vi "Shooter Teleop Handler.vi"() -> ()   [LabVIEW 2025]
uses:
  <vilib>/Rock Robotics/WPI/Joystick/XBox Axes Indexer.ctl
  <vilib>/Rock Robotics/WPI/Joystick/XBox Buttons Indexer.ctl
  Shooter/Implementation/Shooter Modes.ctl
  cc2de0f3-9757-4447-b84a-136412213354.vi
  cac903a5-6411-446e-9ddc-a5b591cf0002.vi
  08590b9f-08c0-4f10-921a-fd0bee2fbc93.vi
  627494dd-781a-424b-80dd-798a3808b72c.vi
  08f81d9b-c70a-4ca4-abda-0492c1fc3297.vi
  <vilib>/Rock Robotics/WPI/Utilities/WPI_GetSetVariantRefNum.vi
  Framework/Robot Global Data.vi
panel:
  in  "Purge Speeds":T1={"Transfer Speed"=-4600.0, "Kicker Speed"=0.95}
  in  "Ticks after shooting":dbl=10.0
  in  "Min Tick":dbl=20.0
  in  "Pre Transfer Speeds":T1={"Transfer Speed"=-1500.0, "Kicker Speed"=-0.4}
  in  "Oh Crap":cluster{"Hood Setpoint":dbl, "Flywheel":dbl}={"Hood Setpoint"=0.0, "Flywheel"=2000.0}
  in  "Tower":cluster{"Hood Setpoint":dbl, "Flywheel":dbl}={"Hood Setpoint"=3.5, "Flywheel"=2370.0}
  in  "A to A (no work)":cluster{"Hood Setpoint":dbl, "Flywheel":dbl}
  in  "C to A Far":cluster{"Hood Setpoint":dbl, "Flywheel":dbl}={"Hood Setpoint"=14.0, "Flywheel"=4600.0}
  in  "C to A Close":cluster{"Hood Setpoint":dbl, "Flywheel":dbl}={"Hood Setpoint"=15.0, "Flywheel"=3200.0}
  in  "Idle Speeds":cluster{"Hood Setpoint":dbl, "Flywheel":dbl}={"Hood Setpoint"=0.0, "Flywheel"=1000.0}
  in  "Transfer Speeds":T1={"Transfer Speed"=4600.0, "Kicker Speed"=0.95}
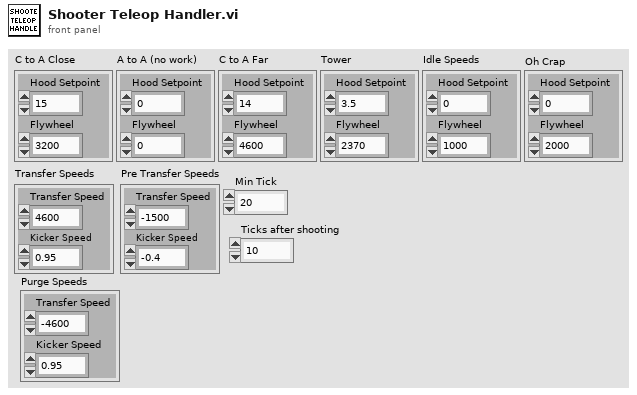
[diagram p1: front panel]
types:
  T1 = cluster{"Transfer Speed":dbl, "Kicker Speed":dbl}
  T2 = typedef "Shooter Modes.ctl" = enum16{"C to A Close", "C to A Far", "A to A", "Tower", "Interp", "Idle"}
  T3 = typedef "XBox Buttons Indexer.ctl" = enum16{"A", "B", "X", "Y", "Left Bumper", "Right Bumper", "Back", "Start", "Left Joystick", "Right Joystick"}
  T4 = typedef "XBox Axes Indexer.ctl" = enum16{"Left X", "Left Y", "Left Trigger", "Right Trigger", "Right X", "Right Y"}
  T5 = typedef "WPI_JoystickDevRef.ctl" = cluster{"Device":T6}
  T6 = typedef "WPI_JoystickDeviceEnum.ctl" = enum16{"USB 0", "USB 1", "USB 2", "USB 3", "USB 4", "USB 5"}
  T7 = cluster{"Hood Setpoint":dbl, "Flywheel Speed":dbl}
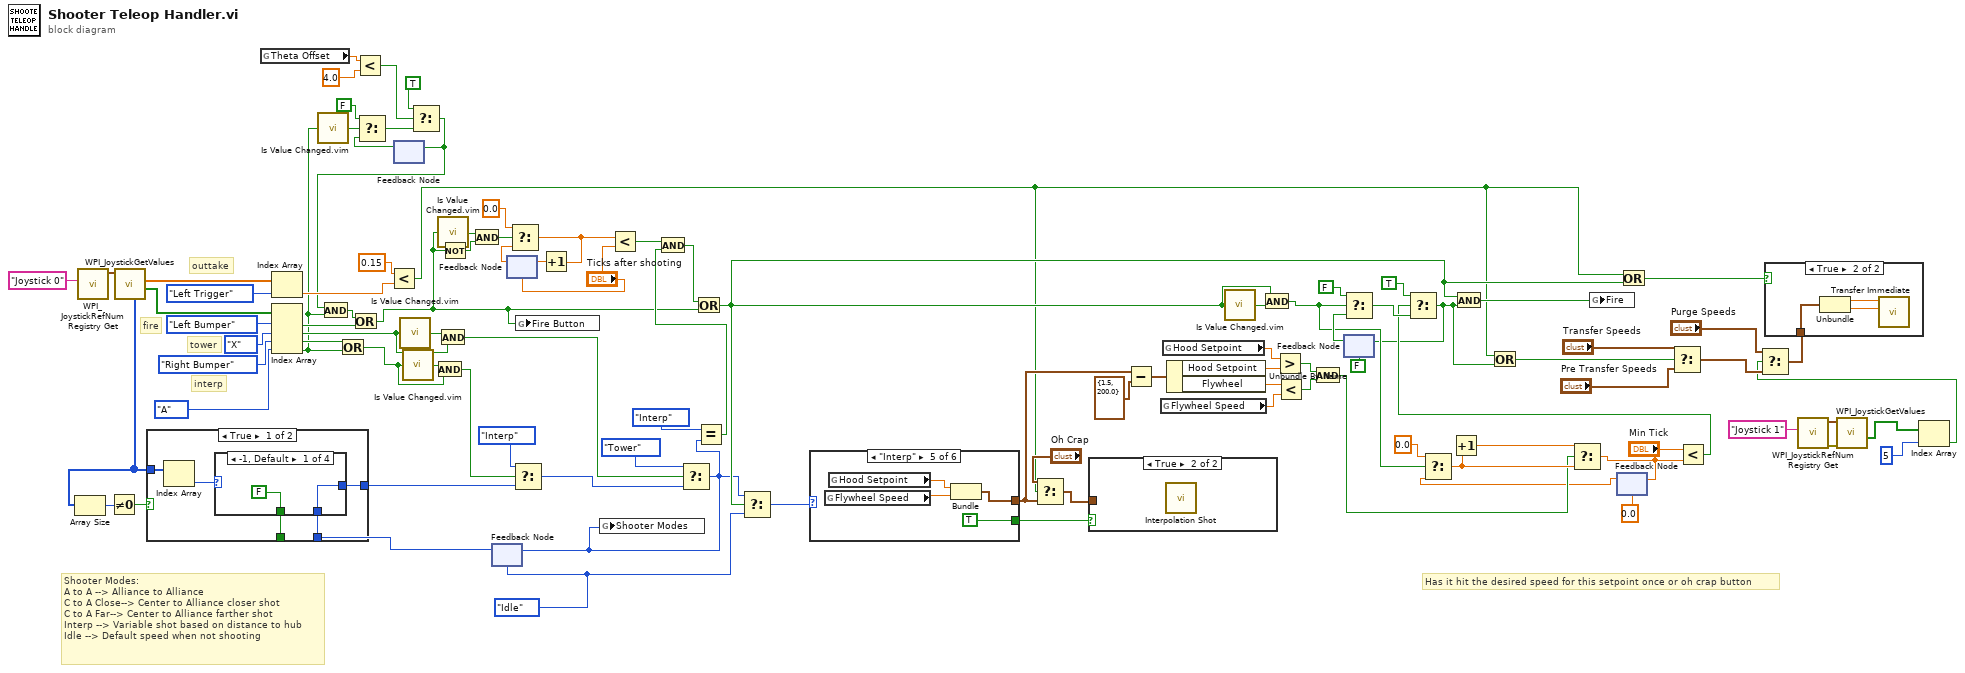
[diagram p0: block diagram]
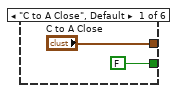
[diagram p3: hidden frame]
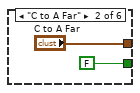
[diagram p4: hidden frame]
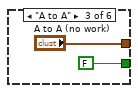
[diagram p5: hidden frame]
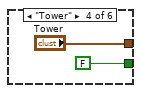
[diagram p6: hidden frame]
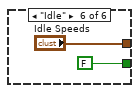
[diagram p7: hidden frame]
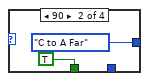
[diagram p8: hidden frame]
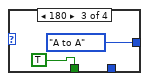
[diagram p9: hidden frame]
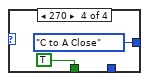
[diagram p10: hidden frame]
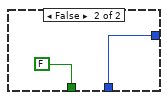
[diagram p11: hidden frame]
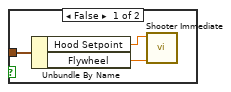
[diagram p12: hidden frame]
diagram:
  w64 = Shooter_Modes."Idle" ("Shooter Modes")
  # "interp"
  # "tower"
  # "Has it hit the desired speed for this setpoint once or oh crap button"
  # "Shooter Modes:\nA to A --> Alliance to Alliance\nC to A Close--> Center to Alliance closer shot\nC to A Far--> Center to Alliance farther shot\nInterp --> Variable shot based on distance to hub\nIdle --> Default speed when not shooting"
  # "outtake"
  # "fire"
  n1 = call <vilib>:"WPI_JoystickRefNum Registry Get.vi"("refnum name"="Joystick 0") -> ("JoystickDevRef"=w98:T5)  [unwired: 1 in, 9 out]
  n2 = call <vilib>:"WPI_JoystickGetValues.vi"("JoystickDevRef"=w98) -> ("Buttons"=w96:bool[], "Axes"=w97:dbl[], "POVs"=w77:i16[])  [unwired: 6 in, 2 out]
  n3 = Array Size(array=w77) -> (size(s)=w93:i32)
  n4 = Not Equal To 0?(x=w93) -> (x != 0?=w76:bool)
  n5 = global read "Robot Global Data.vi" "Theta Offset"() -> (w19:dbl)
  n6 = Index Array(array=w97, index=XBox_Axes_Indexer."Left Trigger" ("XBox Axes")) -> (element=w75:dbl)
  n7 = Index Array(array=w96, index #1=XBox_Buttons_Indexer."Left Bumper" ("XBox Buttons"), index #2=XBox_Buttons_Indexer."X" ("XBox Buttons"), index #3=XBox_Buttons_Indexer."Right Bumper" ("XBox Buttons"), index #4=XBox_Buttons_Indexer."A" ("XBox Buttons")) -> (element #1=w13:bool, element #2=w67:bool, element #3=w27:bool, element #4=w12:bool)
  n8 = call "Is Value Changed.vim"("value"=w12) -> ("changed or first call?"=w21:bool)
  n9 = Or(x=w27, y=w12) -> (x .or. y?=w26:bool)
  n10 = Less?(x=w19, y=4.0) -> (x < y?=w17:bool)
  n11 = Less?(x=0.15, y=w75) -> (x < y?=w23:bool)
  n12 = feedback #1() -> (w15:bool)  [unwired: 1 in]
  n13 = Select(t=FALSE, s=w21, f=w15) -> (s? t:f=w16:bool)
  n14 = call "Is Value Changed.vim"("value"=w67) -> ("changed or first call?"=w68:bool)
  n15 = call "Is Value Changed.vim"("value"=w26) -> ("changed or first call?"=w59:bool)
  n16 = Select(t=TRUE, s=w17, f=w16) -> (s? t:f=w10:bool)
  n17 = And(x=w10, y=w12) -> (x .and. y?=w11:bool)
  n18 = Or(x=w11, y=w13) -> (x .or. y?=w25:bool)
  n19 = feedback-in #1(w10) -> ()
  n20 = And(x=w59, y=w26) -> (x .and. y?=w58:bool)
  n21 = call "Is Value Changed.vim"("value"=w25) -> ("changed or first call?"=w41:bool)
  n22 = And(x=w68, y=w67) -> (x .and. y?=w65:bool)
  n23 = Not(x=w25) -> (.not. x?=w37:bool)
  n24 = And(x=w41, y=w37) -> (x .and. y?=w38:bool)
  n25 = feedback #2(w64) -> (w92:T2)
  n26 = case shown="True" w76 {
    tunnel: w77 -> [w104 _]
    tunnel: [w102 w114] -> w62
    tunnel: w92 -> [w101 w114]
    tunnel: [w100 FALSE ("changed or first call?")] -> _
    frame True {
      n27 = Index Array(array=w104) -> (element=w103:i16)  [unwired: 1 in]
      n28 = case shown="-1, Default" w103 {
        tunnel: [w106 Shooter_Modes."C to A Far" ("Shooter Modes") Shooter_Modes."A to A" ("Shooter Modes") Shooter_Modes."C to A Close" ("Shooter Modes")] -> w102
        tunnel: w101 -> [w106 _ _ _]
        tunnel: [FALSE ("changed or first call?") TRUE ("changed or first call?") TRUE ("changed or first call?") TRUE ("changed or first call?")] -> w100
        frame -1, Default {
        }
        frame 90 {
        }
        frame 180 {
        }
        frame 270 {
        }
      }
    }
    frame False {
    }
  }
  n29 = feedback #3("Ticks after shooting") -> (w40:dbl)
  n30 = Select(t=0.0, s=w38, f=w40) -> (s? t:f=w36:dbl)
  n31 = Select(t=Shooter_Modes."Interp", s=w58, f=w62) -> (s? t:f=w61:T2)
  n32 = global write "Robot Global Data.vi" "Fire Button"(w25) -> ()
  n33 = Increment(x=w36) -> (x+1=w34:dbl)
  n34 = feedback-in #3(w34) -> ()
  n35 = Less?(x=w36, y="Ticks after shooting") -> (x < y?=w32:bool)
  n36 = Select(t=Shooter_Modes."Tower", s=w65, f=w61) -> (s? t:f=w30:T2)
  n37 = feedback-in #2(w30) -> ()
  n38 = global write "Robot Global Data.vi" "Shooter Modes"(w30) -> ()
  n39 = Equal?(x=Shooter_Modes."Interp", y=w30) -> (x = y?=w28:bool)
  n40 = And(x=w32, y=w28) -> (x .and. y?=w31:bool)
  n41 = Or(x=w31, y=w25) -> (x .or. y?=w35:bool)
  n42 = Select(t=w30, s=w35, f=w64) -> (s? t:f=w83:T2)
  n43 = case shown="\"Interp\"" w83 {
    tunnel: ["C to A Close" "C to A Far" "A to A (no work)" "Tower" w125 "Idle Speeds"] -> w72
    tunnel: [FALSE FALSE FALSE FALSE TRUE FALSE] -> w78
    frame "C to A Close", Default {
    }
    frame "C to A Far" {
    }
    frame "A to A" {
    }
    frame "Tower" {
    }
    frame "Interp" {
      n44 = global read "Robot Global Data.vi" "Flywheel Speed"() -> (w123:dbl)
      n45 = global read "Robot Global Data.vi" "Hood Setpoint"() -> (w124:dbl)
      n46 = Bundle("Hood Setpoint"=w124, "Flywheel Speed"=w123) -> (w125:T7)  [unwired: 1 in]
    }
    frame "Idle" {
    }
  }
  n47 = Select(t="Oh Crap", s=w23, f=w72) -> (s? t:f=w73:cluster{"Hood Setpoint":dbl, "Flywheel":dbl})
  n48 = case shown="True" w78 {
    tunnel: w73 -> [w129 _]
    frame False {
      n49 = Unbundle By Name(w129) -> ("Hood Setpoint"=w130:dbl, "Flywheel"=w131:dbl)
      n50 = call "Shooter Immediate.vi"("Flywheel Setpoint"=w131, "Hood Setpoint"=w130) -> ()  [unwired: 7 in, 1 out]
    }
    frame True {
      n51 = call "Interpolation Shot.vi"() -> ()  [unwired: 11 in, 1 out]
    }
  }
  n52 = Subtract(x=w72, y=cluster{"Hood Setpoint":dbl, "Flywheel":dbl} {"Hood Setpoint"=1.5, "Flywheel"=200.0}) -> (x-y=w91:cluster{"Hood Setpoint":dbl, "Flywheel":dbl})
  n53 = global read "Robot Global Data.vi" "Flywheel Speed"() -> (w84:dbl)
  n54 = global read "Robot Global Data.vi" "Hood Setpoint"() -> (w85:dbl)
  n55 = Unbundle By Name(w91) -> ("Hood Setpoint"=w89:dbl, "Flywheel"=w88:dbl)
  n56 = call "Is Value Changed.vim"("value"=w35) -> ("changed or first call?"=w52:bool)
  n57 = And(x=w35, y=w52) -> (x .and. y?=w44:bool)
  n58 = Greater?(x=w85, y=w89) -> (0:w86:bool)
  n59 = Less?(x=w88, y=w84) -> (x < y?=w87:bool)
  n60 = And(x=w86, y=w87) -> (x .and. y?=w45:bool)
  n61 = feedback #4(FALSE) -> (w79:bool)
  n62 = Select(t=FALSE, s=w44, f=w79) -> (s? t:f=w80:bool)
  n63 = feedback #5(0.0 ("t")) -> (w42:dbl)
  n64 = Select(t=0.0, s=w44, f=w42) -> (s? t:f=w46:dbl)
  n65 = Increment(x=w46) -> (x+1=w47:dbl)
  n66 = Select(t=w47, s=w45, f=w46) -> (s? t:f=w43:dbl)
  n67 = feedback-in #5(w43) -> ()
  n68 = Or(x=w23, y=w35) -> (x .or. y?=w55:bool)
  n69 = Less?(x="Min Tick", y=w43) -> (x < y?=w48:bool)
  n70 = Select(t=TRUE, s=w48, f=w80) -> (s? t:f=w24:bool)
  n71 = feedback-in #4(w24) -> ()
  n72 = And(x=w35, y=w24) -> (x .and. y?=w70:bool)
  n73 = Or(x=w23, y=w24) -> (x .or. y?=w22:bool)
  n74 = global write "Robot Global Data.vi" "Fire"(w70) -> ()
  n75 = Select(t="Transfer Speeds", s=w22, f="Pre Transfer Speeds") -> (s? t:f=w3:T1)
  n76 = call <vilib>:"WPI_JoystickRefNum Registry Get.vi"("refnum name"="Joystick 1") -> ("error out"=w7:errorcluster, "JoystickDevRef"=w8:T5)  [unwired: 1 in, 8 out]
  n77 = call <vilib>:"WPI_JoystickGetValues.vi"("error in (no error)"=w7, "JoystickDevRef"=w8) -> ("Buttons"=w6:bool[])  [unwired: 5 in, 4 out]
  n78 = Index Array(array=w6, index=5) -> (element=w2:bool)
  n79 = Select(t="Purge Speeds", s=w2, f=w3) -> (s? t:f=w4:T1)
  n80 = case shown="True" w55 {
    tunnel: w4 -> [_ w132]
    frame False {
    }
    frame True {
      n81 = Unbundle(w132) -> ("Transfer Speed"=w133:dbl, "Kicker Speed"=w134:dbl)
      n82 = call "Transfer Immediate.vi"("Kicker Speed"=w134, "Transfer Speed"=w133) -> ()  [unwired: 9 in, 1 out]
    }
  }
